vi "3D Controller Position Test.vi"() -> ()   [LabVIEW 2023, in "FCC 3D Controller for BS.lvlib"]
uses:
  FCC 3D Controller for BS.lvlib
panel:
  in  "Stop":bool
  out "Waveform Chart":dbl(graph)
  out "Position Info":T1
  in  "VISA resource name":refnum<visa-resource-name>
  in  "error in (no error)":errorcluster
  in  "Axis Index":i32
  in  "Target Angle":dbl
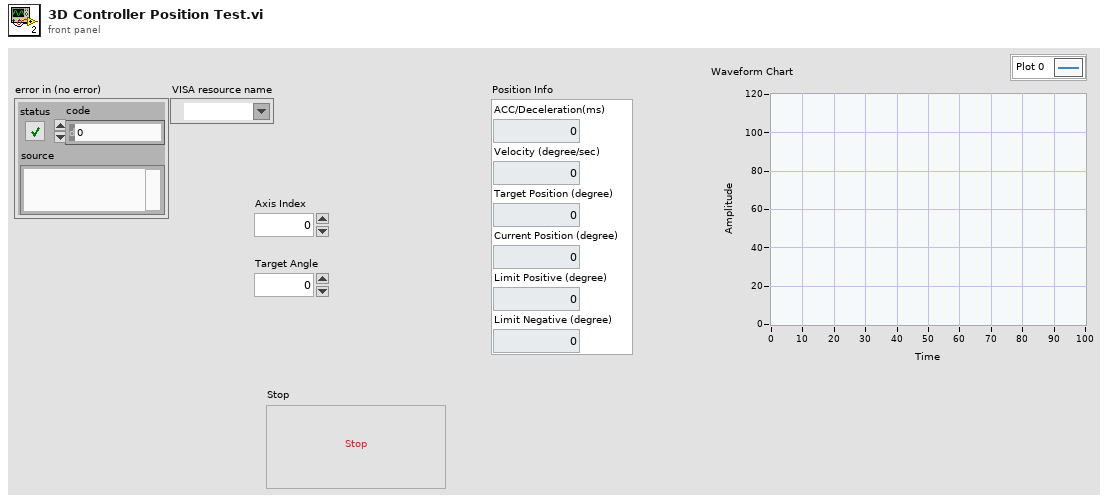
[diagram p1: front panel]
types:
  T1 = cluster{"ACC/Deceleration(ms)":dbl, "Velocity (degree/sec)":dbl, "Target Position (degree)":dbl, "Current Position (degree)":dbl, "Limit Positive (degree)":dbl, "Limit Negative (degree)":dbl}
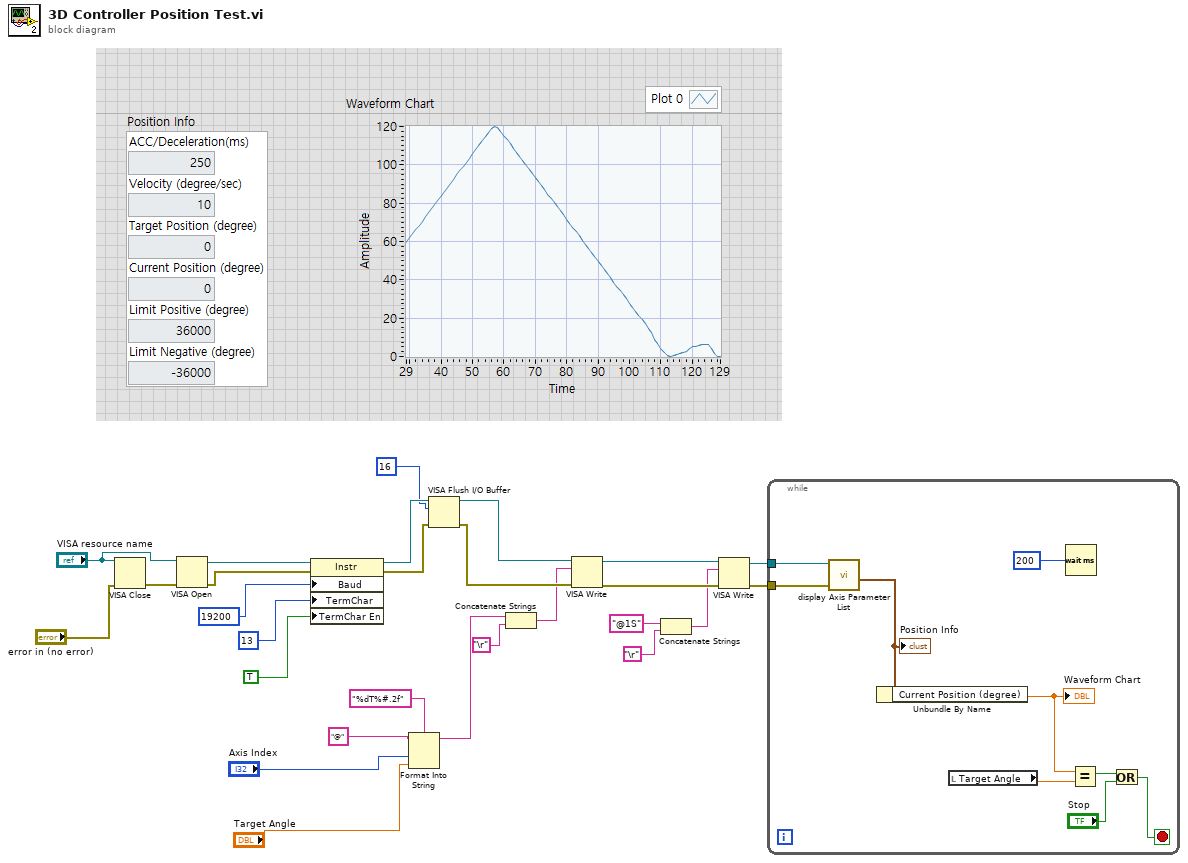
[diagram p0: block diagram]
diagram:
  n1 = VISA Close(VISA resource name="VISA resource name", error in (no error)="error in (no error)") -> (error out=w22:errorcluster)
  n2 = VISA Open(error in (no error)=w22, VISA resource name="VISA resource name") -> (VISA resource name=w20:refnum<visa-resource-name>, error out=w18:errorcluster)  [unwired: 3 in]
  n3 = property class="Instr"(reference=w20, error in=w18, "Baud"=u32 19200 ("Serial Settings:Baud Rate"), "TermChar"=u8 13 ("Message Based Settings:Termination Character"), "TermChar En"=TRUE ("Message Based Settings:Termination Character Enable")) -> (reference out=w14:refnum<visa-resource-name>, error out=w12:errorcluster)
  n4 = Format Into String(format string="%dT%#.2f", initial string="@", "Axis Index", "Target Angle") -> (resulting string=w4:string)  [unwired: 1 in, 1 out]
  n5 = VISA Flush I/O Buffer(VISA resource name=w14, mask (16)=u16 16, error in (no error)=w12) -> (VISA resource name out=w13:refnum<visa-resource-name>, error out=w11:errorcluster)
  n6 = Concatenate Strings(w4, "\r") -> (w2:string)
  n7 = VISA Write(VISA resource name=w13, write buffer=w2, error in (no error)=w11) -> (VISA resource name out=w9:refnum<visa-resource-name>, error out=w8:errorcluster)  [unwired: 1 out]
  n8 = Concatenate Strings("@1S" ("write buffer"), "\r") -> (w1:string)
  n9 = VISA Write(VISA resource name=w9, write buffer=w1, error in (no error)=w8) -> (VISA resource name out=w6:refnum<visa-resource-name>, error out=w5:errorcluster)  [unwired: 1 out]
  n10 = while {
    tunnel: w6 -> [w35]
    tunnel: w5 -> [w34]
    stop <- w29 stop-if-true
    n11 = call "display Axis Parameter List.vi"("error in (no error)"=w34, "VISA resource name"=w35) -> ("Position Info"=w36:T1)  [unwired: 7 in, 2 out]
    "Position Info" <- w36
    n12 = Unbundle By Name(w36) -> ("Current Position (degree)"=w32:dbl)
    "Waveform Chart" <- w32
    n13 = local read "Target Angle"() -> (w33:dbl)
    n14 = Wait (ms)(milliseconds to wait=u32 200) -> ()  [unwired: 1 out]
    n15 = Equal?(x=w32, y=w33) -> (x = y?=w31:bool)
    n16 = Or(x=w31, y="Stop") -> (x .or. y?=w29:bool)
  }
